vi "VIH Dialog - Settings.vi"() -> (0 "OK out":bool)   [LabVIEW 2014]
doc: "::: VI Helpeks :::\nCopyright (c) 2000-2026 Konstantin Shifershteyn. All rights reserved."
uses:
  <vilib>/Utility/miscctls.llb/LVRowAndColumnUnsignedTypeDef.ctl
  _VIH Support Library.llb/VIH Utility - MENU - Create Menu (String).vi
panel:
  in  "Tab Control":enum32{"General", "Edit Programs", "System"}(tab)
  in  "ShowQuickTips":bool caption="Show quick tips at startup"
  in  "FastLoadVI":bool caption="Use fast method to load VIs"
  in  "EdCust_Use":bool caption="Use this file association"
  in  "EdCust_Program":path caption="Program file name or full path"
  in  "EdCust_Extensions":string caption="File Extensions (separate extensions with spaces)"
  in  "EdCustList":i32(listbox) caption="Edit program associations"
  out "Associated path":path
  in  "%AssociationCheck":bool caption="Check VIHelpeks Project File type association"
  in  "%AssociationSet":bool caption="Associate VIHelpeks Project File type"
  out "VIHRUN Associated":bool caption="VIHelpeks Project File is associated"
  in  "%OK":bool
  in  "%Cancel":bool
  # "*) Fast load method might significantly improve speed of loading VIs with many sub-VIs, especially for VIs saved in LabVIEW version other than currently running.\n\n*) Fast load method is available in LabVIEW 2011 and later.\nIt is experimental method. Turn it off if you meet errors or improper results while generating help."
  # "*) If you have several instances of VI Helpeks installed for different LabVIEW versions, no matter which instance is associated. When you open a project using file type association, the most appropriate LabVIEW version is choosen (similar way as when you open a VI from the Windows Explorer)."
  # "*) In order to perform project file type association in Windows 7/8/10/11, LabVIEW should be started with the Run as administrator option (see Windows help for details)."
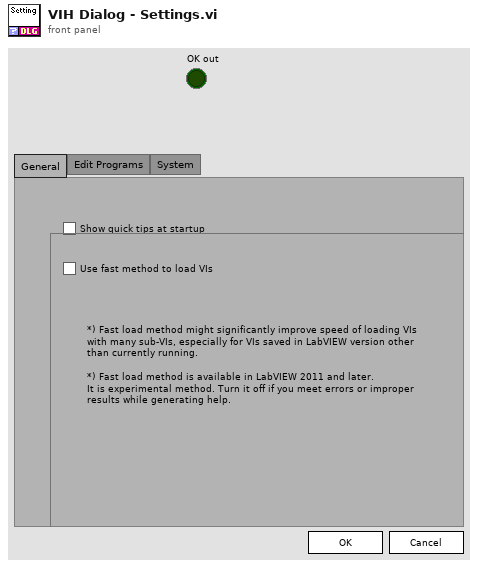
[diagram p1: front panel]
types:
  T1 = cluster{"ShowQuickTips":bool, "NextQuickTip":i32, "FastLoadVI":bool, "EditPrgs ":cluster{"FileExtension":string, "CustProgram":path, "UseCustPrg":bool}[]}
  T2 = typedef "LVRowAndColumnUnsignedTypeDef.ctl" = cluster{"Row":u32, "Column":u32}
  T3 = typedef "LVPoint32TypeDef.ctl" = cluster{"Horizontal":i32, "Vertical":i32}
  T4 = typedef "LVRowAndColumnTypeDef.ctl" = cluster{"Row":i32, "Column":i32}
  T5 = typedef "eventvkey.ctl" = enum16{"ASCII", "Enter", "Return", "Shift", "Ctrl", "Alt", "Cmd", "Opt", "Caps", "NumLock", "Clear", "Break", "Up", "Down", "Left", "Right", "Insert", "Delete", "Home", "End", "PageUp", "PageDown", "Escape", "Help", "Pause", "ScrollLock", "F1", "F2", "F3", "F4", "F5", "F6", "F7", "F8", "F9", "F10", "F11", "F12", "F13", "F14", "F15", "F16", "F17", "F18", "F19", "F20", "F21", "F22", "F23", "F24", "Play", "VolumeUp", "VolumeDown", "Mute", "Two Byte Char"}
  T6 = cluster{"Shift":bool, "Ctrl":bool, "Alt":bool, "Cmd":bool, "Opt":bool}
  T7 = cluster{"FileExtension":string, "CustProgram":path, "UseCustPrg":bool}[]
  T8 = cluster{"FileExtension":string, "CustProgram":path, "UseCustPrg":bool}
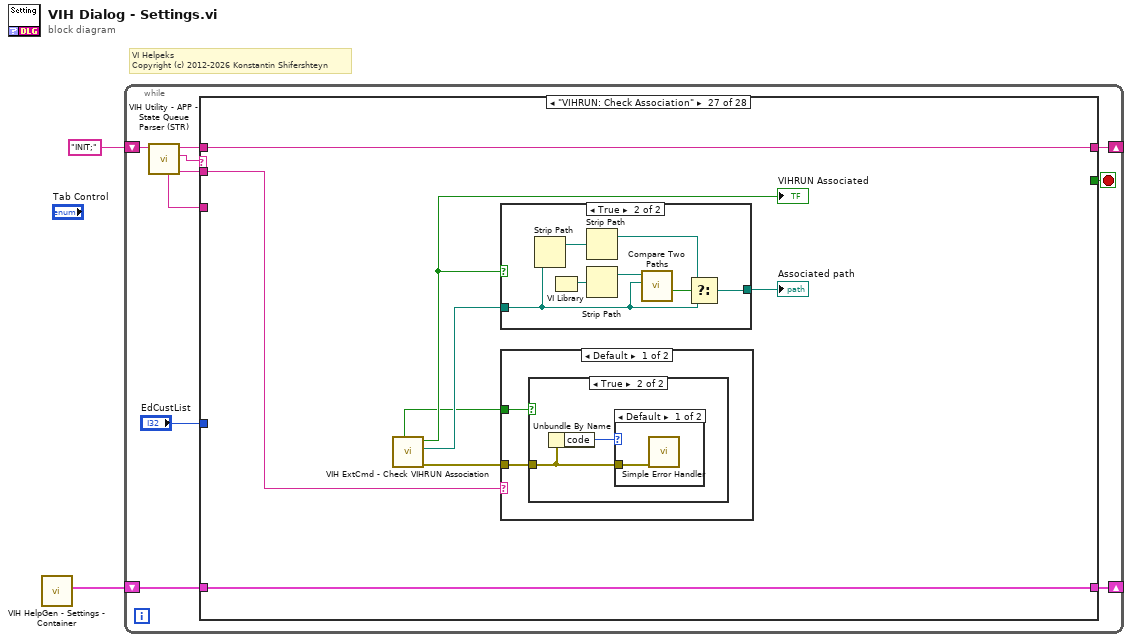
[diagram p0: block diagram]
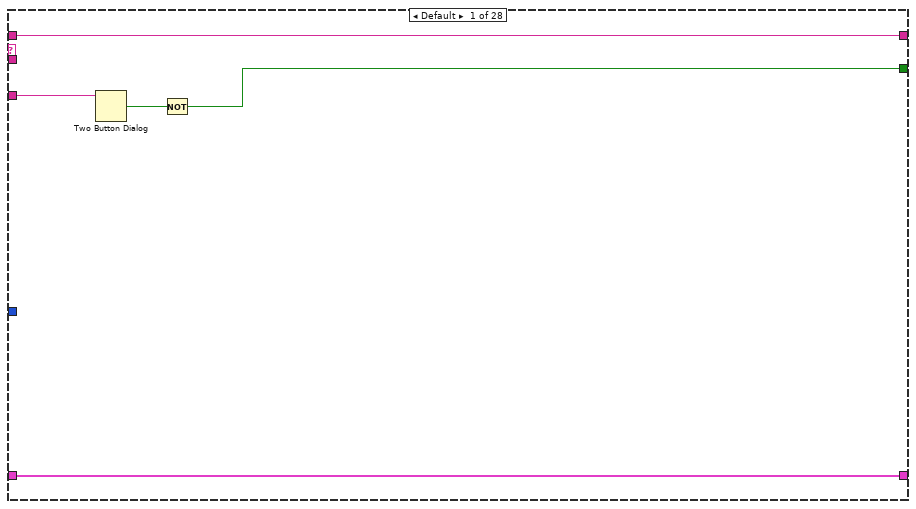
[diagram p2: hidden frame]
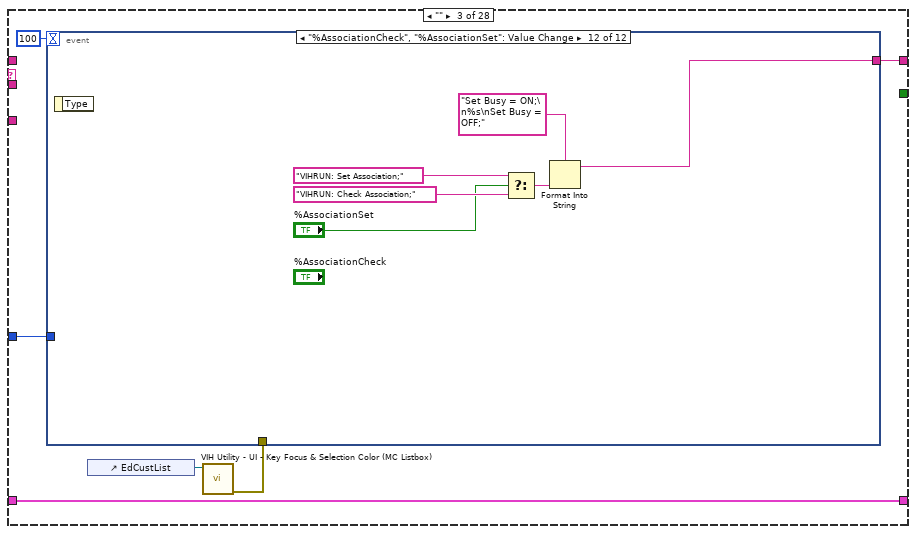
[diagram p4: hidden frame]
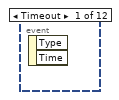
[diagram p5: hidden frame]
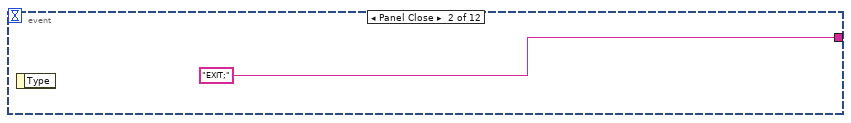
[diagram p6: hidden frame]
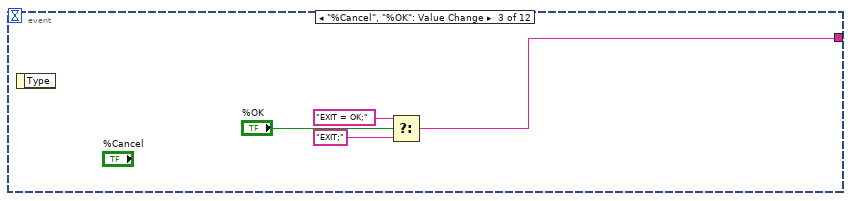
[diagram p7: hidden frame]
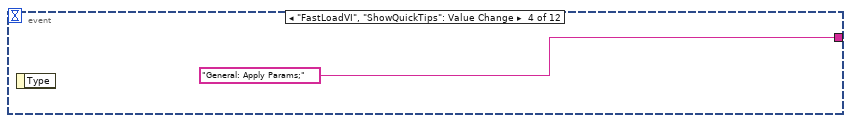
[diagram p8: hidden frame]
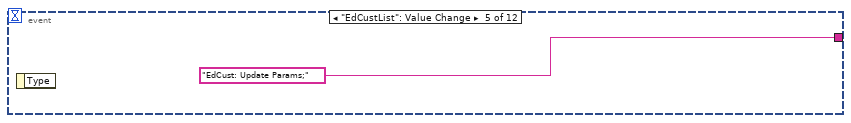
[diagram p9: hidden frame]
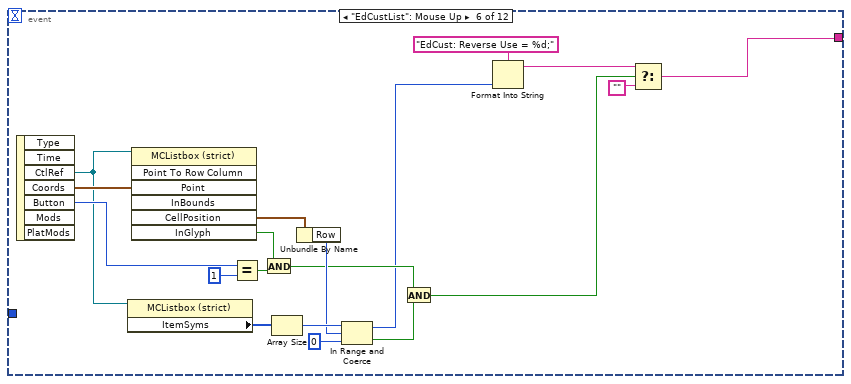
[diagram p10: hidden frame]
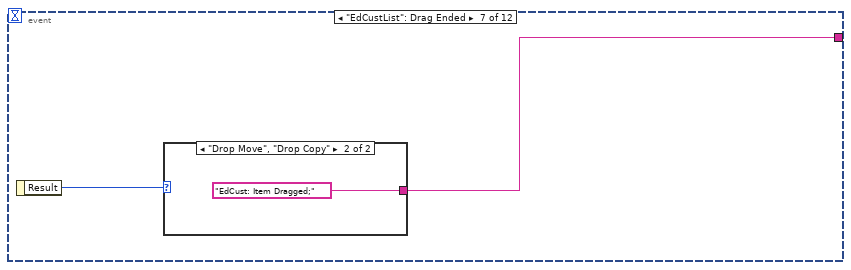
[diagram p11: hidden frame]
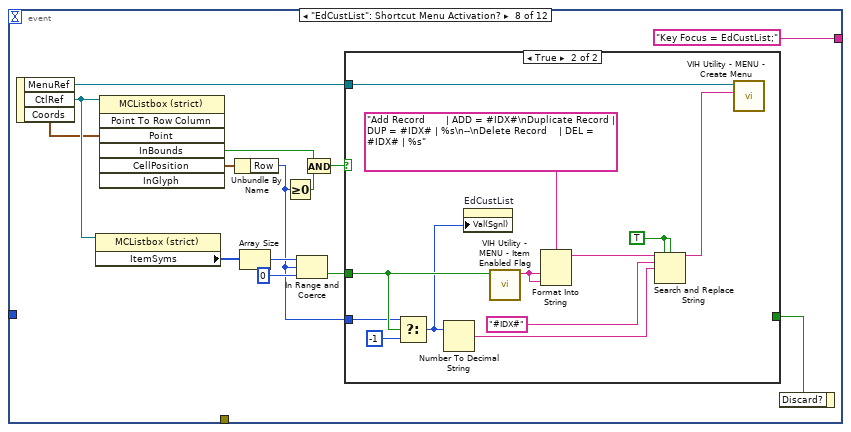
[diagram p13: hidden frame]
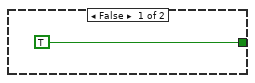
[diagram p14: hidden frame]
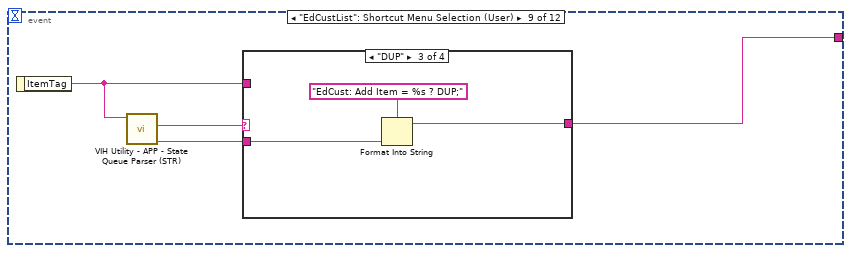
[diagram p15: hidden frame]
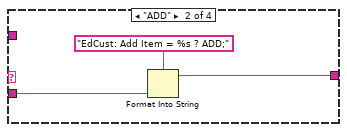
[diagram p17: hidden frame]
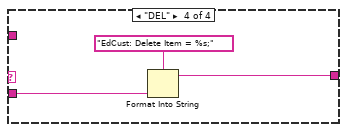
[diagram p18: hidden frame]
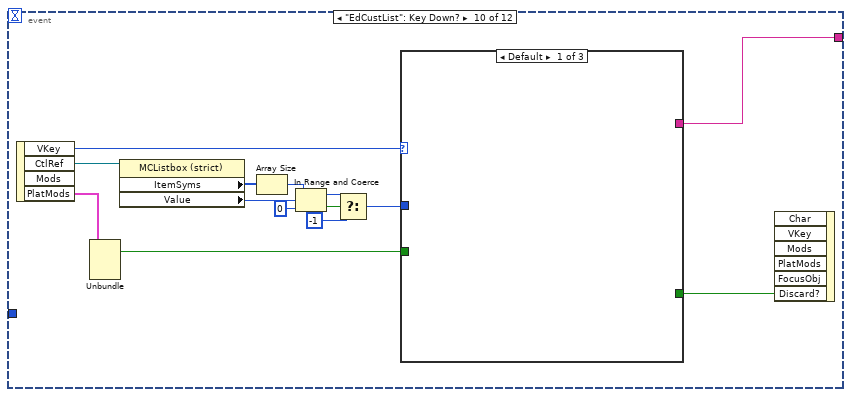
[diagram p19: hidden frame]
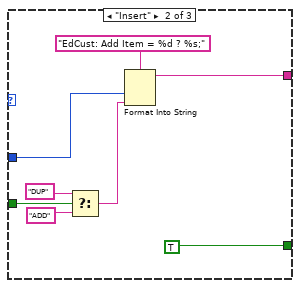
[diagram p20: hidden frame]
diagram:
  # "VI Helpeks\nCopyright (c) 2012-2026 Konstantin Shifershteyn"
  n1 = call "VIH HelpGen - Settings - Container.vi"() -> ("Settings out"=w1:T1)  [unwired: 10 in, 1 out]
  n2 = while {
    shift-right: [w8] -> _
    shift-left: "INIT;" -> [w12]
    shift-right: [w4] -> _
    shift-left: w1 -> [w6]
    stop <- w7 stop-if-true
    n3 = call "VIH Utility - APP - State Queue Parser (STR).vi"("input queue"=w12) -> ("state parameters"=w5:string, "state"=w11:string, "remained queue"=w9:string, "complete state specifier"=w10:string)  [unwired: 5 in]
    n4 = case shown="\"VIHRUN: Check Association\"" w11 {
      tunnel: w10 -> [w17 _ _ _ _ _ _ _ _ _ _ _ _ _ _ _ _ _ _ _ _ _ _ _ _ _ _ _]
      tunnel: w9 -> [w16 w19 _ w132 w149 w154 w162 w165 w169 w175 w178 w186 w189 w193 w198 w200 w216 w223 w238 w248 w256 w277 w295 w314 w340 w348 w356 w373]
      tunnel: [w16 w19 w25 w132 w138 w151 w162 w165 w167 w175 w178 w186 w189 w193 w198 w200 w216 w223 w238 w240 w250 w271 w292 w311 w337 w348 w356 w370] -> w8
      tunnel: [w14 _ _ _ _ _ TRUE _ _ _ _ _ _ _ _ _ _ _ _ _ _ _ _ _ _ _ _ _] -> w7
      tunnel: w6 -> [w13 w18 w24 w131 w141 w153 w161 w164 w168 w174 w177 w187 w188 w192 w197 w199 w215 w222 w237 w247 w255 w276 w294 w313 w339 w347 w355 w372]
      tunnel: w5 -> [_ _ _ _ _ w155 _ _ _ _ w176 w185 _ _ _ _ _ _ _ _ w253 w274 _ w308 w334 _ w353 _]
      tunnel: [w13 w18 w24 w131 w140 w153 w161 w164 w168 w174 w177 w187 w188 w192 w196 w199 w215 w222 w237 w247 w254 w275 w293 w312 w338 w347 w355 w372] -> w4
      tunnel: "EdCustList" -> [_ _ w23 _ _ _ _ _ _ _ _ _ _ _ _ _ w210 _ _ w242 _ _ _ _ _ _ _ _]
      frame Default {
        n5 = Two Button Dialog(message=w17) -> (T button?=w15:bool)  [unwired: 2 in]
        n6 = Not(x=w15) -> (.not. x?=w14:bool)
      }
      frame "#" {
      }
      frame "" {
        n7 = control-ref of="EdCustList"() -> (w21:refnum<vi>)
        n8 = call "VIH Utility - UI - Key Focus & Selection Color (MC Listbox).vi"("MCListbox Refnum"=w21) -> ("error out"=w20:errorcluster)  [unwired: 8 in, 2 out]
        n9 = event shown="[11] \"%AssociationCheck\", \"%AssociationSet\": Value Change" {
          selector: _ -> [_ _ _ _ _ _ _ _ _ _ _ _]
          dyn-events: _ -> [_ _ _ _ _ _ _ _ _ _ _ _]
          timeout: 100 -> [_ _ _ _ _ _ _ _ _ _ _ _]
          tunnel: [_ "EXIT;" w27 "General: Apply Params;" "EdCust: Update Params;" w39 w52 "Key Focus = EdCustList;" w83 w97 w122 w129] -> w25
          tunnel: w23 -> [_ _ _ _ _ _ _ _ _ _ w123 _]
          tunnel: w20 -> [_ _ _ _ _ _ _ _ _ _ _ _]
          event Timeout {
            n10 = event-data() -> ()  [unwired: 1 in, 2 out]
          }
          event Panel Close {
            n11 = event-data() -> ()  [unwired: 1 in, 1 out]
          }
          event "%Cancel", "%OK": Value Change {
            n12 = event-data() -> ()  [unwired: 1 in, 1 out]
            n13 = Select(t="EXIT = OK;", s="%OK", f="EXIT;") -> (s? t:f=w27:string)
          }
          event "FastLoadVI", "ShowQuickTips": Value Change {
            n14 = event-data() -> ()  [unwired: 1 in, 1 out]
          }
          event "EdCustList": Value Change {
            n15 = event-data() -> ()  [unwired: 1 in, 1 out]
          }
          event "EdCustList": Mouse Up {
            n16 = event-data() -> ("CtlRef"=w45:refnum<vi>, "Coords"=w51:T3, "Button"=w49:u16)  [unwired: 1 in, 4 out]
            n17 = property class="MCListbox (strict)"(reference=w45) -> ("ItemSyms"=w44:i32[])  [unwired: 1 in, 2 out]
            n18 = invoke class="MCListbox (strict)" method="Point To Row Column"(reference=w45, "Point"=w51) -> ("CellPosition"=w46:T4, "InGlyph"=w50:bool)  [unwired: 5 in, 5 out]
            n19 = Equal?(x=w49, y=u16 1) -> (x = y?=w47:bool)
            n20 = And(x=w50, y=w47) -> (x .and. y?=w38:bool)
            n21 = Array Size(array=w44) -> (size(s)=w43:i32)
            n22 = Unbundle By Name(w46) -> ("Row"=w42:i32)
            n23 = In Range and Coerce(upper limit=w43, x=w42, lower limit=0) -> (coerced(x)=w35:i32, In Range?=w37:bool)
            n24 = And(x=w38, y=w37) -> (x .and. y?=w36:bool)
            n25 = Format Into String(format string="EdCust: Reverse Use = %d;", w35) -> (resulting string=w33:string)  [unwired: 2 in, 1 out]
            n26 = Select(t=w33, s=w36, f="") -> (s? t:f=w39:string)
          }
          event "EdCustList": Drag Ended {
            n27 = event-data() -> ("Result"=w53:enum16{"Drop Cancel", "Drop Move", "Drop Copy"})  [unwired: 1 in]
            n28 = case shown="\"Drop Move\", \"Drop Copy\"" w53 {
              tunnel: [_ "EdCust: Item Dragged;"] -> w52
              frame "Drop Cancel" {
              }
              frame "Drop Move", "Drop Copy" {
              }
            }
          }
          event "EdCustList": Shortcut Menu Activation? {
            n29 = event-data() -> ("MenuRef"=w57:refnum<k9>, "CtlRef"=w67:refnum<vi>, "Coords"=w63:T3)  [unwired: 1 in]
            n30 = property class="MCListbox (strict)"(reference=w67) -> ("ItemSyms"=w66:i32[])  [unwired: 1 in, 2 out]
            n31 = invoke class="MCListbox (strict)" method="Point To Row Column"(reference=w67, "Point"=w63) -> ("InBounds"=w61:bool, "CellPosition"=w68:T4)  [unwired: 5 in, 5 out]
            n32 = Unbundle By Name(w68) -> ("Row"=w55:i32)
            n33 = Array Size(array=w66) -> (size(s)=w65:i32)
            n34 = Greater Or Equal To 0?(x=w55) -> (x >= 0?=w60:bool)
            n35 = In Range and Coerce(upper limit=w65, x=w55, lower limit=0) -> (In Range?=w56:bool)  [unwired: 1 out]
            n36 = And(x=w61, y=w60) -> (x .and. y?=w59:bool)
            n37 = case shown="True" w59 {
              tunnel: [TRUE _] -> w58
              tunnel: w57 -> [_ w81]
              tunnel: w56 -> [_ w74]
              tunnel: w55 -> [_ w73]
              frame False {
              }
              frame True {
                w77 = TRUE
                n38 = Select(t=w73, s=w74, f=-1) -> (s? t:f=w70:i32)
                n39 = Number To Decimal String(number=w70) -> (decimal integer string=w71:string)  [unwired: 1 in]
                n40 = property on="EdCustList" class="MCListbox (strict)"("Val(Sgnl)"=w70) -> ()  [unwired: 2 in, 2 out]
                n41 = call "VIH Utility - MENU - Item Enabled Flag.vi"("Enable?"=w74) -> ("Disable flag"=w79:string)  [unwired: 10 in]
                n42 = Format Into String(format string="Add Record       | ADD = #IDX#\nDuplicate Record | DUP = #IDX# | %s\n--\nDelete Record    | DEL = #IDX# | %s", w79, w79) -> (resulting string=w78:string)  [unwired: 2 in, 1 out]
                n43 = Search and Replace String(replace all?=w77, case sensitive?=w77, input string=w78, search string="#IDX#", replace string=w71) -> (result string=w76:string)  [unwired: 3 in, 3 out]
                n44 = call-poly "VIH Utility - MENU - Create Menu.vi"("Menu Description"=w76, "menu"=w81) -> ()  [unwired: 8 in, 2 out]
              }
            }
            n45 = event-data("Discard?"=w58) -> ()  [unwired: 1 in, 1 out]
          }
          event "EdCustList": Shortcut Menu Selection (User) {
            n46 = event-data() -> ("ItemTag"=w82:string)  [unwired: 1 in]
            n47 = call "VIH Utility - APP - State Queue Parser (STR).vi"("input queue"=w82) -> ("state parameters"=w84:string, "state"=w85:string)  [unwired: 5 in, 2 out]
            n48 = case shown="\"DUP\"" w85 {
              tunnel: w84 -> [_ w88 w91 w94]
              tunnel: [w86 w87 w90 w93] -> w83
              tunnel: w82 -> [w86 _ _ _]
              frame Default {
              }
              frame "ADD" {
                n49 = Format Into String(format string="EdCust: Add Item = %s ? ADD;", w88) -> (resulting string=w87:string)  [unwired: 2 in, 1 out]
              }
              frame "DUP" {
                n50 = Format Into String(format string="EdCust: Add Item = %s ? DUP;", w91) -> (resulting string=w90:string)  [unwired: 2 in, 1 out]
              }
              frame "DEL" {
                n51 = Format Into String(format string="EdCust: Delete Item = %s;", w94) -> (resulting string=w93:string)  [unwired: 2 in, 1 out]
              }
            }
          }
          event "EdCustList": Key Down? {
            n52 = event-data() -> ("VKey"=w108:T5, "CtlRef"=w107:refnum<vi>, "PlatMods"=w109:T6)  [unwired: 1 in, 1 out]
            n53 = Unbundle(w109) -> ("Ctrl"=w98:bool)  [unwired: 4 out]
            n54 = property class="MCListbox (strict)"(reference=w107) -> ("ItemSyms"=w105:i32[], "Value"=w106:i32)  [unwired: 1 in, 2 out]
            n55 = Array Size(array=w105) -> (size(s)=w104:i32)
            n56 = In Range and Coerce(upper limit=w104, x=w106, lower limit=0) -> (coerced(x)=w101:i32, In Range?=w102:bool)
            n57 = Select(t=w101, s=w102, f=-1) -> (s? t:f=w99:i32)
            n58 = case shown="Default" w108 {
              tunnel: [_ w116 w120] -> w97
              tunnel: w99 -> [_ w115 w119]
              tunnel: w98 -> [_ w114 _]
              tunnel: [_ TRUE TRUE] -> w96
              frame Default {
              }
              frame "Insert" {
                n59 = Select(t="DUP", s=w114, f="ADD") -> (s? t:f=w111:string)
                n60 = Format Into String(format string="EdCust: Add Item = %d ? %s;", w115, w111) -> (resulting string=w116:string)  [unwired: 2 in, 1 out]
              }
              frame "Delete" {
                n61 = Format Into String(format string="EdCust: Delete Item = %d;", w119) -> (resulting string=w120:string)  [unwired: 2 in, 1 out]
              }
            }
            n62 = event-data("Discard?"=w96) -> ()  [unwired: 6 in, 1 out]
          }
          event "EdCust_Extensions", "EdCust_Program", "EdCust_Use": Value Change {
            n63 = event-data() -> ()  [unwired: 1 in, 1 out]
            n64 = Format Into String(format string="EdCust: Apply Params = %d;", w123) -> (resulting string=w122:string)  [unwired: 2 in, 1 out]
          }
          event "%AssociationCheck", "%AssociationSet": Value Change {
            n65 = event-data() -> ()  [unwired: 1 in, 1 out]
            n66 = Select(t="VIHRUN: Set Association;", s="%AssociationSet", f="VIHRUN: Check Association;") -> (s? t:f=w126:string)
            n67 = Format Into String(format string="Set Busy = ON;\n%s\nSet Busy = OFF;", w126) -> (resulting string=w129:string)  [unwired: 2 in, 1 out]
          }
        }
      }
      frame "------------------------- 0" {
      }
      frame "INIT" {
        n68 = Unbundle By Name(w141) -> ("FastLoadVI"=w143:bool)
        n69 = call "VIH ExtCmd - Check VIHRUN Existence.vi"() -> ("Exist"=w136:bool, "Implemented"=w134:bool)  [unwired: 7 in, 3 out]
        n70 = call "VIH Utility - UI - Boolean to Control Disable Status.vi"("Status in"=w134) -> ("Control Disable if False"=w133:u8)  [unwired: 3 in, 1 out]
        n71 = call "VIH Utility - UI - Boolean to Control Disable Status.vi"("Status in"=w136) -> ("Control Disable if False"=w135:u8)  [unwired: 3 in, 1 out]
        n72 = property class="App"() -> ("App.Version"=w148:string)  [unwired: 2 in, 2 out]
        n73 = property on="%AssociationSet" class="Bool"("DisabledEnum"=w135) -> ()  [unwired: 2 in, 2 out]
        n74 = property on="%AssociationCheck" class="Bool"("DisabledEnum"=w133) -> ()  [unwired: 2 in, 2 out]
        n75 = Fract/Exp String To Number(string=w148) -> (number=w147:dbl)  [unwired: 3 in, 1 out]
        n76 = Greater Or Equal?(x=w147, y=11.0) -> (x >= y?=w144:bool)
        n77 = call "VIH Utility - UI - Boolean to Control Disable Status.vi"("Status in"=w144) -> ("Control Disable if False"=w145:u8)  [unwired: 3 in, 1 out]
        n78 = Select(t=w143, s=w144, f=FALSE) -> (s? t:f=w139:bool)
        n79 = property on="FastLoadVI" class="Bool (strict)"("DisabledEnum"=w145) -> ()  [unwired: 2 in, 2 out]
        n80 = Bundle By Name(cluster=w141, "FastLoadVI"=w139) -> (w140:T1)
        n81 = Concatenate Strings("Set Busy = ON;\n\nClear Controls;\n\nGeneral: Update Params;\n\nEdCust: Update List;\nEdCust: Show List Selection;\nEdCust: Update Params;\n\nVIHRUN: Check Association = SILENT;\n\nSet Busy = OFF;", w149) -> (w138:string)
      }
      frame "EXIT" {
        n82 = case shown="\"OK\"" w155 {
          tunnel: w153 -> [_ w160]
          tunnel: [_ TRUE] -> w152
          frame Default {
          }
          frame "OK" {
            n83 = call "VIH HelpGen - Settings - Container.vi"("cmd (get)"=enum16{"get", "set", "load", "save"}."set", "Settings in"=w160) -> ("error out"=w159:errorcluster)  [unwired: 8 in, 1 out]
            n84 = call "VIH HelpGen - Settings - Container.vi"("cmd (get)"=enum16{"get", "set", "load", "save"}."save", "error in"=w159) -> ()  [unwired: 8 in, 2 out]
          }
        }
        "OK out" <- w152
        n85 = Concatenate Strings("Clear Controls;\nHALT;", w154) -> (w151:string)
      }
      frame "HALT" {
      }
      frame "------------------------- 1" {
      }
      frame "Control Appearance" {
        n86 = Concatenate Strings("EdCust: Control Appearance;", w169) -> (w167:string)
      }
      frame "Clear Controls" {
        n87 = property on="EdCustList" class="MCListbox (strict)"("TopLeft"=T2 {"Row"=0, "Column"=0} ("Top Left Visible Cell"), "Value"=-1 ("EdCustList"), "ItemNames"=string[][] [] ("Item Names"), "ItemSyms"=i32[] [] ("Item Symbols")) -> ()  [unwired: 2 in, 2 out]
      }
      frame "Key Focus" {
        n88 = case shown="\"EdCust_Extension\"" w176 {
          frame Default {
          }
          frame "EdCustList" {
            n89 = control-ref of="EdCustList"() -> (w180:refnum<vi>)
            n90 = call "VIH Utility - UI - Key Focus & Selection Color (MC Listbox).vi"("F:Test/T:Set Key Focus (F)"=TRUE, "MCListbox Refnum"=w180) -> ()  [unwired: 7 in, 3 out]
          }
          frame "EdCust_Extension" {
            n91 = property on="EdCust_Extensions" class="Str"() -> ("Value"=w182:string)  [unwired: 2 in, 2 out]
            n92 = String Length(string=w182) -> (length=w183:i32)
            n93 = property on="EdCust_Extensions" class="Str"("Text.Selection End"=w183, "Text.Selection Start"=u32 0 ("Text.Selection:Start"), "Key Focus"=TRUE) -> ()  [unwired: 2 in, 2 out]
          }
        }
      }
      frame "Set Busy" {
        n94 = case shown="\"ON\"" w185 {
          frame Default {
            n95 = call <vilib>:"Unset Busy.vi"() -> ()  [unwired: 11 in, 1 out]
          }
          frame "ON" {
            n96 = call <vilib>:"Set Busy.vi"() -> ()  [unwired: 10 in, 2 out]
          }
        }
      }
      frame "------------------------- 2" {
      }
      frame "General: Update Params" {
        n97 = Unbundle By Name(w192) -> ("ShowQuickTips"=w190:bool, "FastLoadVI"=w191:bool)  [unwired: 1 out]
        n98 = property on="ShowQuickTips" class="Bool (strict)"("Value"=w190) -> ()  [unwired: 2 in, 2 out]
        n99 = property on="FastLoadVI" class="Bool (strict)"("Value"=w191) -> ()  [unwired: 2 in, 2 out]
      }
      frame "General: Apply Params" {
        n100 = Bundle By Name(cluster=w197, "ShowQuickTips"="ShowQuickTips", "FastLoadVI"="FastLoadVI") -> (w196:T1)
      }
      frame "------------------------- 3" {
      }
      frame "EdCust: Control Appearance" {
        n101 = Unbundle By Name(w215) -> ("EditPrgs"=w211:T7)
        n102 = Array Size(array=w211) -> (size(s)=w214:i32)
        n103 = In Range and Coerce(upper limit=w214, x=w210, lower limit=0) -> (In Range?=w212:bool)  [unwired: 1 out]
        n104 = call "VIH Utility - UI - Boolean to Control Disable Status.vi"("Status in"=w212) -> ("Control Disable if False"=w203:u8)  [unwired: 3 in, 1 out]
        n105 = Index Array(array=w211, index=w210) -> (element=w209:T8)
        n106 = Unbundle By Name(w209) -> ("FileExtension"=w207:string, "CustProgram"=w208:path)
        n107 = Empty String/Path?(string/path=w207) -> (empty?=w206:bool)
        n108 = Empty String/Path?(string/path=w208) -> (empty?=w205:bool)
        n109 = Or(x=w206, y=w205) -> (x .or. y?=w204:bool)
        n110 = call "VIH Utility - UI - Boolean to Control Disable Status.vi"("Status in"=w204) -> ("Control Disable if True"=w202:u8)  [unwired: 3 in, 1 out]
        n111 = Max & Min(x=w202, y=w203) -> (max(x,y)=w201:u8)  [unwired: 1 out]
        n112 = property on="EdCust_Use" class="Bool (strict)"("DisabledEnum"=w201) -> ()  [unwired: 2 in, 2 out]
        n113 = property on="EdCust_Extensions" class="Str"("DisabledEnum"=w203) -> ()  [unwired: 2 in, 2 out]
        n114 = property on="EdCust_Program" class="Path"("DisabledEnum"=w203) -> ()  [unwired: 2 in, 2 out]
      }
      frame "EdCust: Update List" {
        n115 = Unbundle By Name(w222) -> ("EditPrgs"=w221:T7)
        n116 = for {
          tunnel: w221 -> [w233] mode=indexing
          tunnel: [w226] -> w220 mode=indexing
          tunnel: [w225] -> w219 mode=indexing
          n117 = Unbundle By Name(w233) -> ("FileExtension"=w232:string, "CustProgram"=w231:path, "UseCustPrg"=w229:bool)
          n118 = Path To String(path=w231) -> (string=w230:string)
          n119 = Build Array("", w232, w230) -> (w226:string[])
          n120 = Select(t=38, s=w229, f=37) -> (s? t:f=w225:i32)
        }
        n121 = call "VIH Utility - UI - Drag and Drop Supporter (w Symbol Indices).vi"("Cmd"=enum16{"make symbols", "test D'n'D"}."make symbols", "Item Symbols"=w219) -> ("Item Symbols out"=w218:i32[])  [unwired: 7 in, 2 out]
        n122 = property on="EdCustList" class="MCListbox (strict)"("ItemNames"=w220, "ItemSyms"=w218) -> ()  [unwired: 2 in, 2 out]
      }
      frame "EdCust: Show List Selection" {
        n123 = control-ref of="EdCustList"() -> (w236:refnum<vi>)
        n124 = property class="MCListbox (strict)"(reference=w236) -> (reference out=w235:refnum<vi>, "Value"=w234:i32)  [unwired: 1 in, 1 out]
        n125 = call "VIH Utility - UI - Make Row Visible (MC Listbox).vi"("Row"=w234, "MC Listbox Refnum"=w235) -> ()  [unwired: 8 in, 2 out]
      }
      frame "EdCust: Update Params" {
        n126 = Unbundle By Name(w247) -> ("EditPrgs"=w241:T7)
        n127 = Index Array(array=w241, index=w242) -> (element=w246:T8)
        n128 = Unbundle By Name(w246) -> ("FileExtension"=w245:string, "CustProgram"=w244:path, "UseCustPrg"=w243:bool)
        n129 = property on="EdCust_Extensions" class="Str"("Value"=w245) -> ()  [unwired: 2 in, 2 out]
        n130 = property on="EdCust_Program" class="Path"("Value"=w244) -> ()  [unwired: 2 in, 2 out]
        n131 = property on="EdCust_Use" class="Bool (strict)"("Value"=w243) -> ()  [unwired: 2 in, 2 out]
        n132 = Concatenate Strings("EdCust: Control Appearance;", w248) -> (w240:string)
      }
      frame "EdCust: Apply Params" {
        n133 = Decimal String To Number(string=w253, default (0L)=-1 ("default (0 I32)")) -> (number=w251:i32)  [unwired: 1 in, 1 out]
        n134 = in-place {
          in-place-border: w251 -> [w257]
          n135 = in-place-cluster #1(w255) -> ("EditPrgs"=w259:T7)
          n136 = in-place {
            n137 = in-place-array #2(w259, w257) -> (w269:T8)
            n138 = call <vilib>:"Trim Whitespace.vi"("string"="EdCust_Extensions") -> ("trimmed string"=w264:string)  [unwired: 1 in]
            n139 = Empty String/Path?(string/path=w264) -> (empty?=w266:bool)
            n140 = Empty String/Path?(string/path="EdCust_Program") -> (empty?=w265:bool)
            n141 = Not Or(1:w265, 2:w266) -> (0:w262:bool)
            n142 = And(x=w262, y="EdCust_Use") -> (x .and. y?=w260:bool)
            n143 = Bundle By Name(cluster=w269, "FileExtension"=w264, "CustProgram"="EdCust_Program", "UseCustPrg"=w260) -> (w268:T8)
            n144 = in-place-array #2(w268) -> (w258:T7)  [unwired: 1 out]
          }
          n145 = in-place-cluster #1("EditPrgs"=w258) -> (w254:T1)
        }
        n146 = Concatenate Strings("EdCust: Update List;\nEdCust: Update Params;", w256) -> (w250:string)
      }
      frame "EdCust: Reverse Use" {
        n147 = Decimal String To Number(string=w274, default (0L)=-1 ("default (0 I32)")) -> (number=w272:i32)  [unwired: 1 in, 1 out]
        n148 = in-place {
          in-place-border: w272 -> [w278]
          n149 = in-place-cluster #3(w276) -> ("EditPrgs"=w280:T7)
          n150 = in-place {
            n151 = in-place-array #4(w280, w278) -> (w282:T8)
            n152 = in-place {
              n153 = in-place-cluster #5(w282) -> ("FileExtension"=w287:string, "CustProgram"=w286:path, "UseCustPrg"=w290:bool)
              n154 = Empty String/Path?(string/path=w287) -> (empty?=w289:bool)
              n155 = Empty String/Path?(string/path=w286) -> (empty?=w288:bool)
              n156 = Not Or(1:w288, 2:w289) -> (0:w285:bool)
              n157 = Not(x=w290) -> (.not. x?=w284:bool)
              n158 = And(x=w285, y=w284) -> (x .and. y?=w283:bool)
              n159 = in-place-cluster #5("FileExtension"=w287, "CustProgram"=w286, "UseCustPrg"=w283) -> (w281:T8)
            }
            n160 = in-place-array #4(w281) -> (w279:T7)  [unwired: 1 out]
          }
          n161 = in-place-cluster #3("EditPrgs"=w279) -> (w275:T1)
        }
        n162 = Concatenate Strings("EdCust: Update List;\nEdCust: Update Params;", w277) -> (w271:string)
      }
      frame "EdCust: Item Dragged" {
        n163 = in-place {
          n164 = in-place-cluster #6(w294) -> ("EditPrgs"=w298:T7)
          n165 = property on="EdCustList" class="MCListbox (strict)"() -> ("ItemSyms"=w299:i32[])  [unwired: 2 in, 2 out]
          n166 = call "VIH Utility - UI - Drag and Drop Supporter (w Symbol Indices).vi"("Cmd"=enum16{"make symbols", "test D'n'D"}."test D'n'D", "Item Symbols"=w299) -> ("indices"=w297:i32[])  [unwired: 7 in, 2 out]
          n167 = for {
            tunnel: w298 -> [w303]
            tunnel: w297 -> [w302] mode=indexing
            tunnel: [w301] -> w296 mode=indexing
            n168 = Index Array(array=w303, index=w302) -> (element=w301:T8)
          }
          n169 = in-place-cluster #6("EditPrgs"=w296) -> (w293:T1)
        }
        n170 = Concatenate Strings("EdCust: Update List;\nEdCust: Update Params;", w295) -> (w292:string)
      }
      frame "EdCust: Add Item" {
        n171 = Match Pattern(string=w308, regular expression="\\s*\\?\\s*") -> (before substring=w306:string, after substring=w304:string)  [unwired: 1 in, 2 out]
        n172 = Decimal String To Number(string=w306, default (0L)=-1 ("default (0 I32)")) -> (number=w305:i32)  [unwired: 1 in, 1 out]
        n173 = in-place {
          in-place-border: w305 -> [w316]
          in-place-border: w304 -> [w324]
          n174 = in-place-cluster #7(w313) -> ("EditPrgs"=w317:T7)
          n175 = Greater Or Equal To 0?(x=w316) -> (x >= 0?=w322:bool)
          n176 = Array Size(array=w317) -> (size(s)=w320:i32)
          n177 = Index Array(array=w317, index=w316) -> (element=w315:T8)
          n178 = Increment(x=w316) -> (x+1=w321:i32)
          n179 = Select(t=w321, s=w322, f=w320) -> (s? t:f=w319:i32)
          n180 = case shown="\"ADD\", Default" w324 {
            tunnel: [w328 w330] -> w323
            tunnel: w315 -> [w329 w330]
            frame "ADD", Default {
              n181 = Bundle By Name(cluster=w329, "FileExtension"="", "CustProgram"=path "", "UseCustPrg"=FALSE) -> (w328:T8)
            }
            frame "DUP" {
            }
          }
          n182 = Insert Into Array(array=w317, index=w319, new element=w323) -> (w318:T7)
          n183 = local write "EdCustList"(w319) -> ()
          n184 = in-place-cluster #7("EditPrgs"=w318) -> (w312:T1)
        }
        n185 = Concatenate Strings("EdCust: Update List;\nEdCust: Show List Selection;\nEdCust: Update Params;\n\nKey Focus = EdCust_Extension;", w314) -> (w311:string)
      }
      frame "EdCust: Delete Item" {
        n186 = Match Pattern(string=w334, regular expression="\\s*\\?\\s*") -> (before substring=w332:string)  [unwired: 1 in, 3 out]
        n187 = Decimal String To Number(string=w332, default (0L)=-1 ("default (0 I32)")) -> (number=w331:i32)  [unwired: 1 in, 1 out]
        n188 = in-place {
          in-place-border: w331 -> [w341]
          n189 = in-place-cluster #8(w339) -> ("EditPrgs"=w346:T7)
          n190 = Delete From Array(array=w346, index=w341) -> (array with subset deleted=w345:T7)  [unwired: 1 in, 1 out]
          n191 = Array Size(array=w345) -> (size(s)=w344:i32)
          n192 = Decrement(x=w344) -> (x-1=w343:i32)
          n193 = Max & Min(x=w343, y=w341) -> (min(x,y)=w342:i32)  [unwired: 1 out]
          n194 = local write "EdCustList"(w342) -> ()
          n195 = in-place-cluster #8("EditPrgs"=w345) -> (w338:T1)
        }
        n196 = Concatenate Strings("EdCust: Update List;\nEdCust: Show List Selection;\nEdCust: Update Params;", w340) -> (w337:string)
      }
      frame "------------------------- 4" {
      }
      frame "VIHRUN: Check Association" {
        n197 = call "VIH ExtCmd - Check VIHRUN Association.vi"() -> ("error out"=w354:errorcluster, "VIHRUN path"=w352:path, "Associated"=w350:bool, "Implemented"=w349:bool)  [unwired: 7 in, 1 out]
        "VIHRUN Associated" <- w350
        n198 = case shown="True" w350 {
          tunnel: w352 -> [_ w358]
          tunnel: [_ w363] -> w351
          frame False {
          }
          frame True {
            n199 = Strip Path(path=w358) -> (stripped path=w362:path)  [unwired: 1 out]
            n200 = VI Library() -> (path=w359:path)
            n201 = Strip Path(path=w362) -> (stripped path=w361:path)  [unwired: 1 out]
            n202 = Strip Path(path=w359) -> (stripped path=w360:path)  [unwired: 1 out]
            n203 = call <vilib>:"Compare Two Paths.vi"("Path 2"=w358, "Path 1"=w360) -> ("Path 2 Relative to Path 1?"=w357:bool)  [unwired: 6 in, 3 out]
            n204 = Select(t=w361, s=w357, f=w358) -> (s? t:f=w363:path)
          }
        }
        "Associated path" <- w351
        n205 = case shown="Default" w353 {
          tunnel: w354 -> [w365 _]
          tunnel: w349 -> [w364 _]
          frame Default {
            n206 = case shown="True" w364 {
              tunnel: w365 -> [_ w367]
              frame False {
              }
              frame True {
                n207 = Unbundle By Name(w367) -> ("code"=w366:i32)
                n208 = case shown="Default" w366 {
                  tunnel: w367 -> [w368 _]
                  frame Default {
                    n209 = call <vilib>:"Simple Error Handler.vi"("error in (no error)"=w368) -> ()  [unwired: 4 in, 5 out]
                  }
                  frame -603 {
                  }
                }
              }
            }
          }
          frame "SILENT" {
          }
        }
      }
      frame "VIHRUN: Set Association" {
        n210 = call "VIH ExtCmd - Associate VIHRUN.vi"() -> ("error out"=w371:errorcluster)  [unwired: 11 in]
        n211 = call <vilib>:"Simple Error Handler.vi"("error in (no error)"=w371) -> ()  [unwired: 4 in, 5 out]
        n212 = Concatenate Strings("VIHRUN: Check Association = SILENT;", w373) -> (w370:string)
      }
    }
  }
